vi "Launcher.vi"() -> ()   [LabVIEW 2021, in "Echo Broadcast with External Client.lvlib"]
uses:
  Echo Broadcast with External Client.lvlib
  WebSocket Actor/WebSocket Connection/Keepalive.ctl
  WS Server/WS Server.lvclass
  C:/Program Files/National Instruments/LabVIEW 2021/vi.lib/ActorFramework/Actor/Actor.lvclass
  WebSocket Actor/WebSocket Server Manager/WebSocket Server Manager.lvclass
  WebSocket Actor/WebSocket Server Manager/WebSocket Server Manager.lvclass/WebSocket Server Manager.ctl
  WS Server/WS Server.lvclass/WS Server.ctl
  WebSocket Actor/WebSocket Server Manager/Write Keepalive.vi
  WS Server/properties/Write WebSocket Server Manager Enqueuer.vi
  <vilib>/ActorFramework/Actor/Actor.lvclass
  WebSocket Actor/WebSocket Connection/WebSocket Connection.lvclass
panel:
  in  "Keepalive":T1={"Enabled"=TRUE, "Ping Interval (ms)"=25000, "Ping Timeout (ms)"=20000}
  out "error out":errorcluster
  # "In this example the main actor allows the user to launch WebSocket Server Actors with user defined listener settings by means of the Server Manager Actor Infrastructure.  The user will then be able to add services to such server that will echo back the data sent by the client. You an use any client such as for example the one implemented as Chrome extension downloadable here \nhttps://chrome.google.com/webstore/detail/simple-websocket-client/pfdhoblngboilpfeibdedpjgfnlcodoo\n\nyou need to connect to the ws://localhost:6163/echo WebSocket"
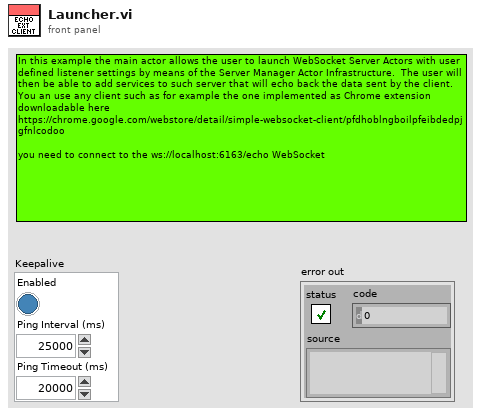
[diagram p1: front panel]
types:
  T1 = typedef "WebSocket Actors.lvlib/WebSocket Connection.lvclass/Keepalive.ctl" = cluster{"Enabled":bool, "Ping Interval (ms)":u32, "Ping Timeout (ms)":u32}
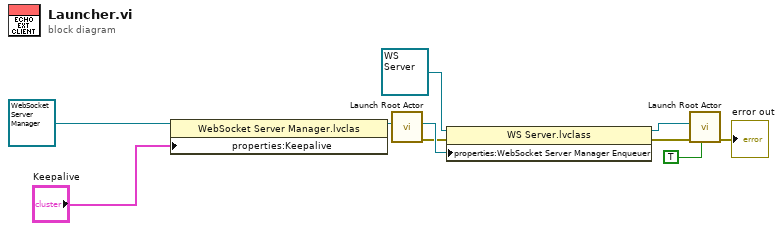
[diagram p0: block diagram]
diagram:
  n1 = property class="WebSocket Server Manager.lvclas"(reference=refnum<class "WebSocket Server Manager.lvclass"> refnum ("WebSocket Actors.lvlib:WebSocket Server Manager.lvclass"), "properties:Keepalive"="Keepalive") -> (reference out=w2:refnum<class "WebSocket Server Manager.lvclass">)  [unwired: 1 in, 1 out]
  n2 = call <vilib>:"Launch Root Actor.vi"("Actor"=w2) -> ("error out"=w4:errorcluster, "Actor's Enqueuer"=w5:refnum<class "Message Enqueuer.lvclass">)  [unwired: 9 in]
  n3 = property class="WS Server.lvclass"(reference=refnum<class "WS Server.lvclass"> refnum ("WS Full LabVIEW Test.lvlib:WS Test Server.lvclass"), error in=w4, "properties:WebSocket Server Manager Enqueuer"=w5) -> (reference out=w6:refnum<class "WS Server.lvclass">, error out=w3:errorcluster)
  n4 = call <vilib>:"Launch Root Actor.vi"("Open Actor Core front panel? (F)"=TRUE, "error in (no error)"=w3, "Actor"=w6) -> ("error out"=→"error out":errorcluster)  [unwired: 7 in, 1 out]
